vi "CSE - Not A CSE RefNum.vi"(0 "CSE RefNum":T1) -> (1 "dynamically opened":bool, 2 "Not a CSE RefNum":bool)   [LabVIEW 2021]
doc: "The VI validates <B>CSE RefNum</B>. Refer to the VI help for more details.\n\n<<B>not a CSE RefNum</B>> indicator returns TRUE if <B>CSE RefNum</B> is not a valid reference to a CSE instance context.\n\n<<B>dynamically opened</B>> indicator returns TRUE if <B>CSE RefNum</B>> is valid and refers to a dynamically created CSE instance context.\n\n::: CalcExpress Toolkit :::\nCopyright (c) 2000-2026 Konstantin Shifershteyn. All rights reserved."
uses:
  CSE Instance RefNum.ctl
  cersrc/celveng32.dll
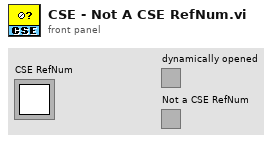
[diagram p1: front panel]
types:
  T1 = typedef "CSE Instance RefNum.ctl" = refnum<k1>
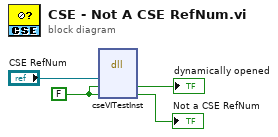
[diagram p0: block diagram]
diagram:
  w3 = FALSE ("not a CE Instance")
  n1 = dll-call lib="C:/LV Projects/CalcExpress 40 LV2021/vi.lib/addons/CalcExpress/cersrc/celveng*.dll" fn="cseVITestInst" ("viCESPTestInst")("iRef"="CSE RefNum", "dynamical"=w3, "erf"=w3) -> ("dynamical"=→"dynamically opened":bool, "erf"=→"Not a CSE RefNum":bool)  [unwired: 5 in, 2 out]
